vi "Serial_Comm.vi"(0 "ESP32_Data":refnum<visa-resource-name>="COM20", 3 "error in":errorcluster) -> (7 "Roll_result":refnum<visa-resource-name>, 10 "error out":errorcluster)   [LabVIEW 2026]
uses:
  <vilib>/Instr/_visa.llb/VISA Configure Serial Port (Instr).vi
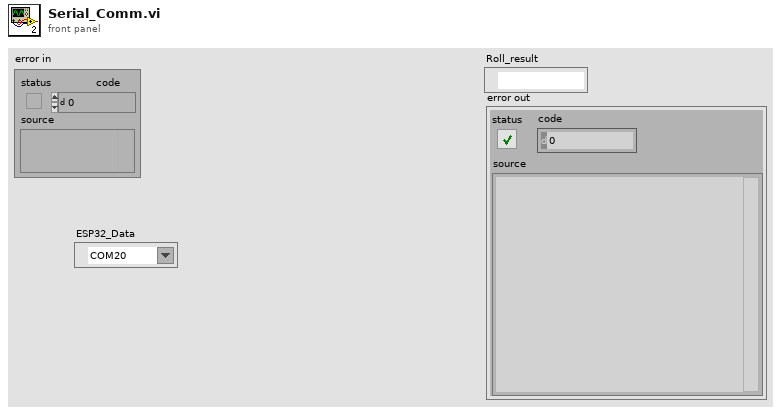
[diagram p1: front panel]
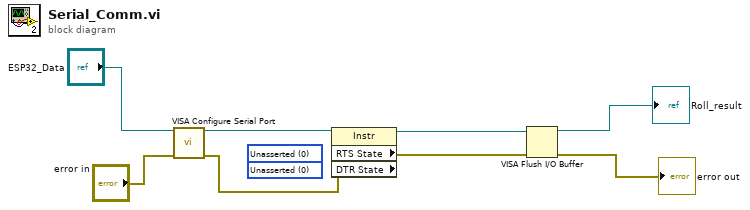
[diagram p0: block diagram]
diagram:
  (unwired) i16 0 items=["Unknown"=-1, "Unasserted"=0, "Asserted"=1] ("Serial Settings:Modem Line Settings:Line DTR State")
  (unwired) i16 0 items=["Unknown"=-1, "Unasserted"=0, "Asserted"=1] ("Serial Settings:Modem Line Settings:Line RTS State")
  n1 = call-poly "VISA Configure Serial Port"("VISA resource name"="ESP32_Data", "error in (no error)"="error in") -> ("VISA resource name out"=w6:refnum<visa-resource-name>, "error out"=w4:errorcluster)  [unwired: 12 in]
  n2 = property class="Instr" props=["RTS State", "DTR State"](reference=w6, error in=w4) -> (reference out=w5:refnum<visa-resource-name>, error out=w3:errorcluster)  [unwired: 2 out]
  n3 = VISA Flush I/O Buffer(VISA resource name=w5, error in (no error)=w3) -> (VISA resource name out=→"Roll_result":refnum<visa-resource-name>, error out=→"error out":errorcluster)  [unwired: 1 in]
